vi "compress.buffer.generated.vi"(9 "start.idx":u8, 10 "buffer.length":u8=8, 11 "buffer":u64[](array[numeric])=[4822678189205111, 0, 0, 0, 0, 0, 0, 0, 0]) -> (2 "buffer.length.out":u8, 3 "buffer.out":u64[](array[numeric]))   [LabVIEW 2020]
doc: "Drop start.idx bytes from the front of buffer and move the remaining buffer.length - start.idx bytes to the top of buffer.out (byte 0 in the MSB of word 0). Rebuilds output words 0..2 (remainders up to 24 bytes) and masks every byte at or beyond the new length, so a remainder longer than one word after an already-complete message is preserved. Replaces compress.buffer.vi, which rebuilt word 0 only."
panel:
  out "Mask 2":u64
  out "Mask 1":u64
  out "Mask 0":u64
  out "Word":u8
  out "Remainder.idx":u8
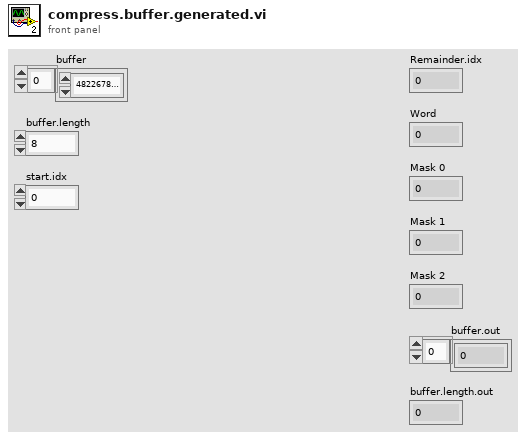
[diagram p1: front panel]
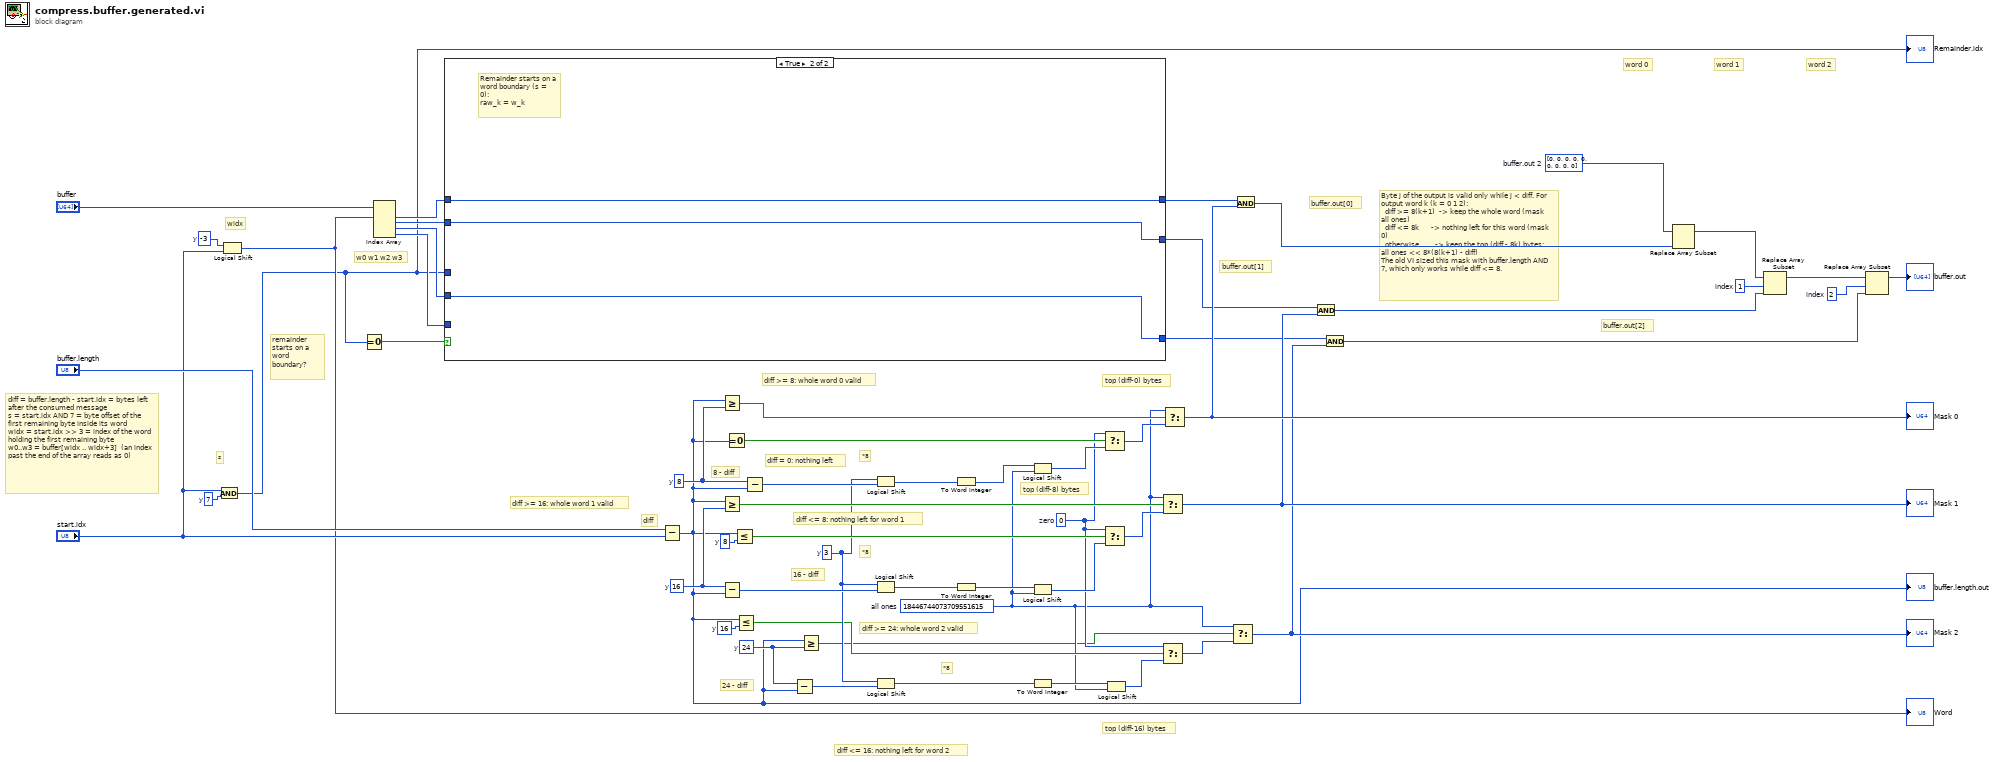
[diagram p0: block diagram]
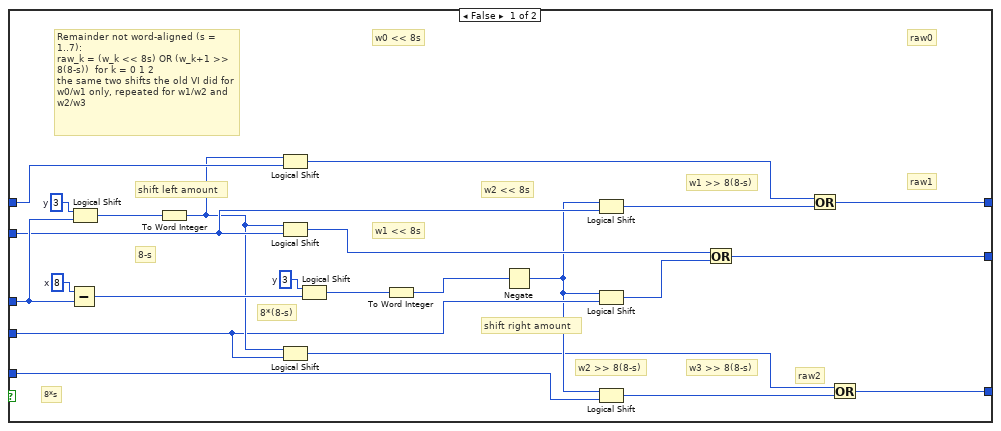
[diagram p2: hidden frame]
diagram:
  w24 = u8 16  # y
  w23 = u8 24  # y
  w35 = u8 8  # y
  w34 = u8 16  # y
  w45 = u8 8  # y
  w4 = 2  # index
  w7 = 1  # index
  w18 = u64 0  # zero
  w22 = i16 3  # y
  w15 = u64 18446744073709551615  # all ones
  w10 = u64[] [0, 0, 0, 0, 0, 0, 0, 0, 0]  # buffer.out 2
  w55 = i16 -3  # y
  w56 = u8 7  # y
  # "word 2"
  # "word 1"
  # "word 0"
  # "buffer.out[2]"
  # "top (diff-16) bytes"
  # "*8"
  # "24 - diff"
  # "diff <= 16: nothing left for word 2"
  # "diff >= 24: whole word 2 valid"
  # "buffer.out[1]"
  # "top (diff-8) bytes"
  # "*8"
  # "16 - diff"
  # "diff <= 8: nothing left for word 1"
  # "diff >= 16: whole word 1 valid"
  # "buffer.out[0]"
  # "top (diff-0) bytes"
  # "*8"
  # "8 - diff"
  # "diff = 0: nothing left"
  # "diff >= 8: whole word 0 valid"
  # "Byte j of the output is valid only while j < diff. For output word k (k = 0 1 2):\n  diff >= 8(k+1)  -> keep the whole word (mask all ones)\n  diff <= 8k      -> nothing left for this word (mask 0)\n  otherwise        -> keep the top (diff - 8k) bytes: all ones << 8*(8(k+1) - diff)\nThe old VI sized this mask with buffer.length AND 7, which only works while diff <= 8."
  # "w0 w1 w2 w3"
  # "remainder starts on a word boundary?"
  # "widx"
  # "s"
  # "diff"
  # "diff = buffer.length - start.idx = bytes left after the consumed message\ns = start.idx AND 7 = byte offset of the first remaining byte inside its word\nwidx = start.idx >> 3 = index of the word holding the first remaining byte\nw0..w3 = buffer[widx .. widx+3]  (an index past the end of the array reads as 0)"
  n1 = And(x="start.idx", y=w56) -> (x .and. y?=w47:u8)
  "Remainder.idx" <- w47
  n2 = Logical Shift(y=w55, x="start.idx") -> (x << y=w52:u8)
  "Word" <- w52
  n3 = Equal To 0?(x=w47) -> (x = 0?=w46:bool)
  n4 = Index Array(array="buffer", index #1=w52) -> (element #1=w51:u64, element #2=w50:u64, element #3=w49:u64, element #4=w48:u64)  [unwired: 3 in]
  n5 = case shown="True" w46 {
    tunnel: w51 -> [w72 w83]
    tunnel: w50 -> [w68 w82]
    tunnel: w49 -> [w63 w81]
    tunnel: w48 -> [w61 _]
    tunnel: w47 -> [w77 _]
    tunnel: [w69 w83] -> w37
    tunnel: [w65 w82] -> w26
    tunnel: [w58 w81] -> w12
    frame False {
      w76 = i16 3  # y
      w78 = u8 8  # x
      w80 = i16 3  # y
      # "raw2"
      # "w3 >> 8(8-s)"
      # "w2 << 8s"
      # "raw1"
      # "w2 >> 8(8-s)"
      # "w1 << 8s"
      # "raw0"
      # "w1 >> 8(8-s)"
      # "w0 << 8s"
      # "shift right amount"
      # "8*(8-s)"
      # "8-s"
      # "shift left amount"
      # "8*s"
      # "Remainder not word-aligned (s = 1..7):\nraw_k = (w_k << 8s) OR (w_k+1 >> 8(8-s))  for k = 0 1 2\nthe same two shifts the old VI did for w0/w1 only, repeated for w1/w2 and w2/w3"
      n6 = Subtract(x=w78, y=w77) -> (x-y=w75:u8)
      n7 = Logical Shift(y=w80, x=w77) -> (x << y=w79:u8)
      n8 = To Word Integer(number=w79) -> (16bit integer=w64:i16)
      n9 = Logical Shift(y=w64, x=w72) -> (x << y=w71:u64)
      n10 = Logical Shift(y=w64, x=w68) -> (x << y=w67:u64)
      n11 = Logical Shift(y=w64, x=w63) -> (x << y=w60:u64)
      n12 = Logical Shift(y=w76, x=w75) -> (x << y=w74:u8)
      n13 = To Word Integer(number=w74) -> (16bit integer=w73:i16)
      n14 = Negate(x=w73) -> (-x=w62:i16)
      n15 = Logical Shift(y=w62, x=w68) -> (x << y=w70:u64)
      n16 = Logical Shift(y=w62, x=w63) -> (x << y=w66:u64)
      n17 = Logical Shift(y=w62, x=w61) -> (x << y=w59:u64)
      n18 = Or(x=w67, y=w66) -> (x .or. y?=w65:u64)
      n19 = Or(x=w71, y=w70) -> (x .or. y?=w69:u64)
      n20 = Or(x=w60, y=w59) -> (x .or. y?=w58:u64)
    }
    frame True {
      # "Remainder starts on a word boundary (s = 0):\nraw_k = w_k"
    }
  }
  n21 = Subtract(x="buffer.length", y="start.idx") -> (x-y=w1:u8)
  "buffer.length.out" <- w1
  n22 = Greater Or Equal?(x=w1, y=w45) -> (x >= y?=w39:bool)
  n23 = Greater Or Equal?(x=w1, y=w34) -> (x >= y?=w28:bool)
  n24 = Subtract(x=w34, y=w1) -> (x-y=w33:u8)
  n25 = Equal To 0?(x=w1) -> (x = 0?=w41:bool)
  n26 = Less Or Equal?(x=w1, y=w35) -> (x <= y?=w30:bool)
  n27 = Less Or Equal?(x=w1, y=w24) -> (x <= y?=w17:bool)
  n28 = Subtract(x=w45, y=w1) -> (x-y=w44:u8)
  n29 = Subtract(x=w23, y=w1) -> (x-y=w21:u8)
  n30 = Greater Or Equal?(x=w1, y=w23) -> (x >= y?=w14:bool)
  n31 = Logical Shift(y=w22, x=w44) -> (x << y=w43:u8)
  n32 = Logical Shift(y=w22, x=w33) -> (x << y=w32:u8)
  n33 = Logical Shift(y=w22, x=w21) -> (x << y=w20:u8)
  n34 = To Word Integer(number=w43) -> (16bit integer=w42:i16)
  n35 = To Word Integer(number=w32) -> (16bit integer=w31:i16)
  n36 = Logical Shift(y=w42, x=w15) -> (x << y=w40:u64)
  n37 = Logical Shift(y=w31, x=w15) -> (x << y=w29:u64)
  n38 = To Word Integer(number=w20) -> (16bit integer=w19:i16)
  n39 = Select(t=w18, s=w41, f=w40) -> (s? t:f=w38:u64)
  n40 = Select(t=w18, s=w30, f=w29) -> (s? t:f=w27:u64)
  n41 = Logical Shift(y=w19, x=w15) -> (x << y=w16:u64)
  n42 = Select(t=w15, s=w28, f=w27) -> (s? t:f=w25:u64)
  "Mask 1" <- w25
  n43 = Select(t=w18, s=w17, f=w16) -> (s? t:f=w13:u64)
  n44 = Select(t=w15, s=w39, f=w38) -> (s? t:f=w36:u64)
  "Mask 0" <- w36
  n45 = Select(t=w15, s=w14, f=w13) -> (s? t:f=w11:u64)
  "Mask 2" <- w11
  n46 = And(x=w37, y=w36) -> (x .and. y?=w9:u64)
  n47 = And(x=w26, y=w25) -> (x .and. y?=w6:u64)
  n48 = And(x=w12, y=w11) -> (x .and. y?=w3:u64)
  n49 = Replace Array Subset(array=w10, new element=w9) -> (w8:u64[])  [unwired: 1 in]
  n50 = Replace Array Subset(array=w8, new element=w6, index=w7) -> (w5:u64[])
  n51 = Replace Array Subset(array=w5, new element=w3, index=w4) -> (→"buffer.out":u64[])
